vi "FuncVI-smatchx.vi"(5 "InstanceRef":T2, 9 "arg list":T1[](array[typedef]) {"num" format="%.2f"}) -> (0 "error out":bool, 3 "result":T1 {"num" format="%.2f"})   [LabVIEW 2021]
doc: "::: CalcExpress Toolkit :::\nCopyright (c) 2000-2026 Konstantin Shifershteyn. All rights reserved."
uses:
  cetypes.llb/CalcExpress Function Argument Info.ctl
  cetypes.llb/CalcExpress Instance RefNum.ctl
panel:
  in  "max arg num":i32=3
  in  "min arg num":i32=2
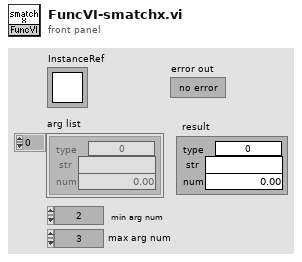
[diagram p1: front panel]
types:
  T1 = typedef "CalcExpress Function Argument Info.ctl" = cluster{"type":u32, "str":string, "num":dbl}
  T2 = typedef "CalcExpress Instance RefNum.ctl" = refnum<k1>
  T3 = cluster{"index":i32, "data type":enum32{"String", "DBL Number", "identifier", "1D Array of DBL", "2D Array of DBL", "CDB Number", "1D Array of CDB", "2D Array of CDB", "1D Array of String", "2D Array of String", "Unknown data type"}, "default num":dbl, "default str":string}
  T4 = enum32{"String", "DBL Number", "identifier", "1D Array of DBL", "2D Array of DBL", "CDB Number", "1D Array of CDB", "2D Array of CDB", "1D Array of String", "2D Array of String", "Unknown data type"}
  T5 = cluster{"index":i32, "any type":i32, "default num":dbl, "default str":string}
  T6 = cluster{"index":i32, "any type":u32, "default num":dbl, "default str":string}[]
  T7 = cluster{"data type":enum32{"String", "DBL Number", "identifier", "1D Array of DBL", "2D Array of DBL", "CDB Number", "1D Array of CDB", "2D Array of CDB", "1D Array of String", "2D Array of String", "Unknown data type"}, "data string":string, "num":dbl}
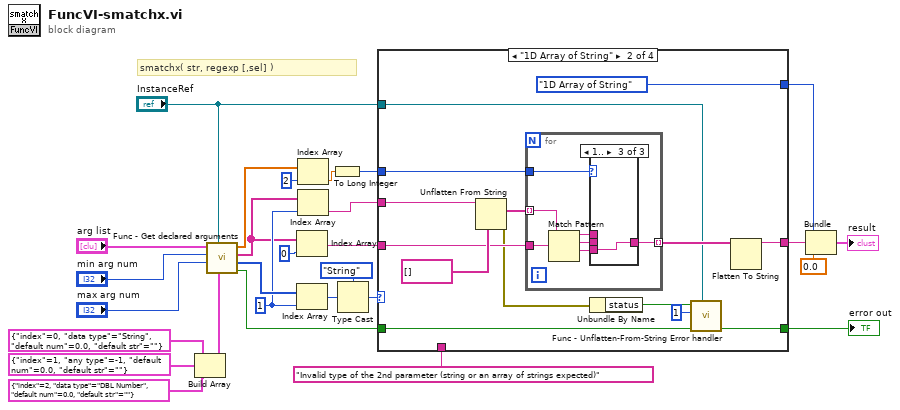
[diagram p0: block diagram]
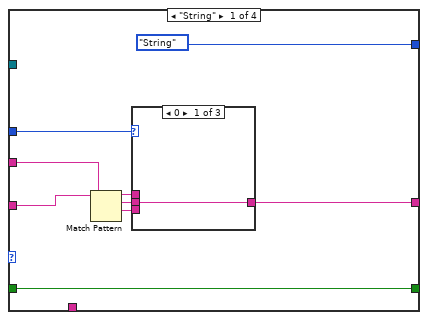
[diagram p2: hidden frame]
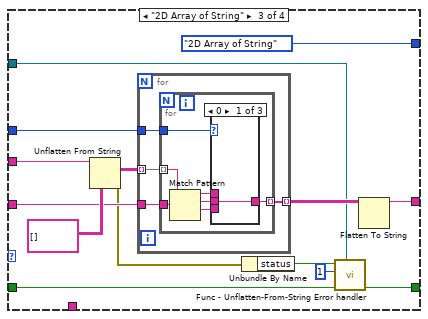
[diagram p7: hidden frame]
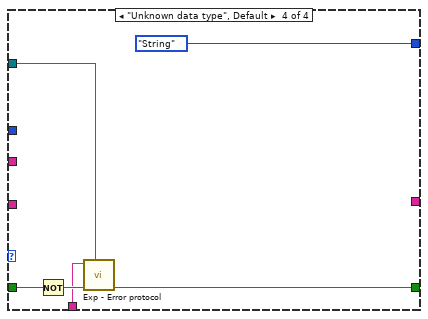
[diagram p10: hidden frame]
diagram:
  w16 = 1
  # "smatchx( str, regexp [,sel] )"
  n1 = Build Array(T3 {"index"=0, "data type"=enum."String", "default num"=0.0, "default str"=""} ("arg descriptor"), T5 {"index"=1, "any type"=-1, "default num"=0.0, "default str"=""} ("arg descriptor"), T3 {"index"=2, "data type"=enum."DBL Number", "default num"=0.0, "default str"=""} ("arg descriptor")) -> (w22:T6)
  n2 = call "Func - Get declared arguments.vi"("arg descriptors"=w22, "InstanceRef"="InstanceRef", "max arg num"="max arg num", "min arg num"="min arg num", "arg list"="arg list") -> ("error out"=w15:bool, "type list"=w17:u32[], "str list"=w11:string[], "num list"=w10:dbl[])  [unwired: 3 in]
  n3 = Index Array(array=w11, index=0) -> (element=w26:string)
  n4 = Index Array(array=w17, index=w16) -> (element=w19:u32)
  n5 = Index Array(array=w10, index=2) -> (element=w25:dbl)
  n6 = Index Array(array=w11, index=w16) -> (element=w18:string)
  n7 = To Long Integer(number=w25) -> (32bit integer=w9:i32)
  n8 = Type Cast(type=T4."String" ("data type"), x=w19) -> (*(type *) &x=w20:T4)
  n9 = case shown="\"1D Array of String\"" w20 {
    tunnel: w18 -> [w29 w44 w77 _]
    tunnel: [w31 w51 w74 _] -> w8
    tunnel: w26 -> [w30 w42 w66 _]
    tunnel: w9 -> [w35 w53 w76 _]
    tunnel: w15 -> [w37 w46 w71 w98]
    tunnel: [w37 w45 w72 w96] -> w14
    tunnel: "Invalid type of the 2nd parameter (string or an array of strings expected)" ("ErrStr") -> [_ _ _ w95]
    tunnel: "InstanceRef" -> [_ w49 w68 w94]
    tunnel: [T4."String" ("data type") T4."1D Array of String" ("data type") T4."2D Array of String" ("data type") T4."String" ("data type")] -> w6
    frame "String" {
      n10 = Match Pattern(string=w30, regular expression=w29) -> (before substring=w32:string, match substring=w34:string, after substring=w33:string)  [unwired: 1 in, 1 out]
      n11 = case shown="0" w35 {
        tunnel: w32 -> [_ w39 _]
        tunnel: w34 -> [w38 _ _]
        tunnel: w33 -> [_ _ w40]
        tunnel: [w38 w39 w40] -> w31
        frame 0 {
        }
        frame ..-1 {
        }
        frame 1.. {
        }
      }
    }
    frame "1D Array of String" {
      n12 = Unflatten From String(type=string[] [], binary string=w44) -> (value=w43:string[], error out=w41:errorcluster)  [unwired: 3 in, 1 out]
      n13 = for {
        tunnel: w53 -> [w61]
        tunnel: [w60] -> w52 mode=indexing
        tunnel: w43 -> [w56] mode=indexing
        tunnel: w42 -> [w55]
        n14 = Match Pattern(string=w55, regular expression=w56) -> (before substring=w57:string, match substring=w59:string, after substring=w58:string)  [unwired: 1 in, 1 out]
        n15 = case shown="1.." w61 {
          tunnel: w57 -> [_ w63 _]
          tunnel: w59 -> [w62 _ _]
          tunnel: w58 -> [_ _ w64]
          tunnel: [w62 w63 w64] -> w60
          frame 0 {
          }
          frame ..-1 {
          }
          frame 1.. {
          }
        }
      }
      n16 = Unbundle By Name(w41) -> ("status"=w48:bool)
      n17 = call "Func - Unflatten-From-String Error handler.vi"("InstanceRef"=w49, "error in"=w46, "argument number"=1, "Unflatten Error status"=w48) -> ("error out"=w45:bool)  [unwired: 5 in]
      n18 = Flatten To String(anything=w52) -> (data string=w51:string)  [unwired: 3 in, 2 out]
    }
    frame "2D Array of String" {
      n19 = Unflatten From String(type=string[][] [], binary string=w77) -> (value=w67:string[][], error out=w65:errorcluster)  [unwired: 3 in, 1 out]
      n20 = for {
        tunnel: w66 -> [w82]
        tunnel: w76 -> [w81]
        tunnel: [w80] -> w75 mode=indexing
        tunnel: w67 -> [w79] mode=indexing
        n21 = for {
          tunnel: w82 -> [w86]
          tunnel: w81 -> [w85]
          tunnel: [w84] -> w80 mode=indexing
          tunnel: w79 -> [w83] mode=indexing
          n22 = Match Pattern(string=w86, regular expression=w83) -> (before substring=w87:string, match substring=w89:string, after substring=w88:string)  [unwired: 1 in, 1 out]
          n23 = case shown="0" w85 {
            tunnel: w87 -> [_ w91 _]
            tunnel: w89 -> [w90 _ _]
            tunnel: w88 -> [_ _ w92]
            tunnel: [w90 w91 w92] -> w84
            frame 0 {
            }
            frame ..-1 {
            }
            frame 1.. {
            }
          }
        }
      }
      n24 = Unbundle By Name(w65) -> ("status"=w70:bool)
      n25 = call "Func - Unflatten-From-String Error handler.vi"("InstanceRef"=w68, "error in"=w71, "argument number"=1, "Unflatten Error status"=w70) -> ("error out"=w72:bool)  [unwired: 5 in]
      n26 = Flatten To String(anything=w75) -> (data string=w74:string)  [unwired: 3 in, 2 out]
    }
    frame "Unknown data type", Default {
      n27 = Not(x=w98) -> (.not. x?=w97:bool)
      n28 = call "Exp - Error protocol.vi"("InstanceRef"=w94, "error in"=w97, "error message in"=w95) -> ("error out"=w96:bool)  [unwired: 5 in, 1 out]
    }
  }
  "error out" <- w14
  n29 = Bundle("data type"=w6, "data string"=w8, "num"=0.0) -> (→"result":T7)  [unwired: 1 in]
